vi "Condition_Editor.vi"(8 "error in (no error)":errorcluster={"status"=FALSE, "code"=0, "source"="\"\""}, 10 "parameter definitions":string, 11 "ConditionNode tree":string) -> (0 "error out":errorcluster={"status"=FALSE, "code"=0, "source"="\"\""}, 2 "status ok":bool, 3 "Validated tree":string)   [LabVIEW 2026]
doc: "INTENT: Build AND/OR expression trees. LOGIC: Build nested operators and compare nodes; show units, quality behavior, reference source."
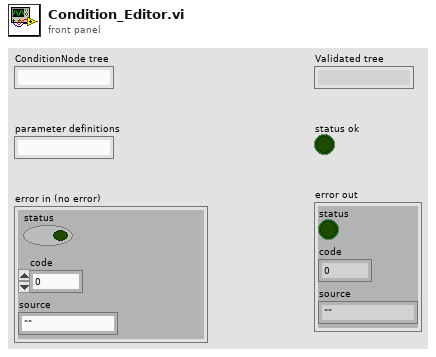
[diagram p1: front panel]
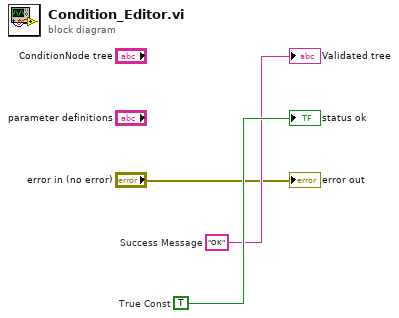
[diagram p0: block diagram]
diagram:
  w3 = TRUE  # True Const
  w2 = "OK"  # Success Message
  "Validated tree" <- w2
  "status ok" <- w3
  "error out" <- "error in (no error)"
